vi "GV_SetGraph.vi"(8 "error in (no error)":errorcluster, 11 "Gviewer in":refnum<class "Gviewer.lvclass">) -> (0 "error out":errorcluster, 3 "Gviewer out":refnum<class "Gviewer.lvclass">)   [LabVIEW 2020, in "Sgraph_lib_V1.lvlib" / "Gviewer.lvclass"]
doc: "Set the Size and Position of the Graph"
uses:
  Gviewer.lvclass
  <vilib>/Utility/miscctls.llb/LVPositionTypeDef.ctl
  <vilib>/Utility/miscctls.llb/LVBoundsTypeDef.ctl
  Gviewer.lvclass/Gviewer.ctl
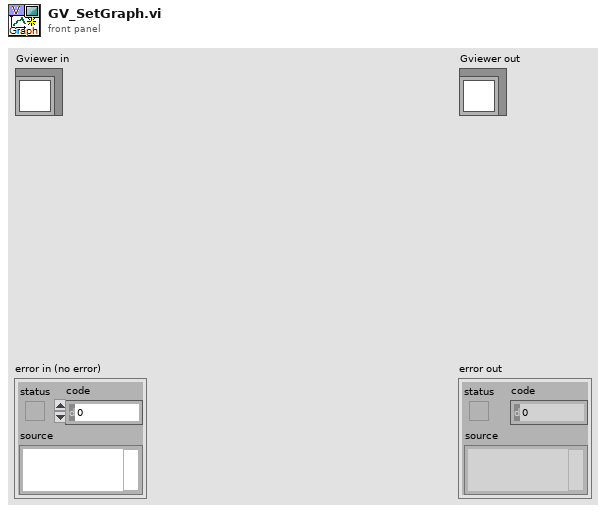
[diagram p1: front panel]
types:
  T1 = typedef "LVBoundsTypeDef.ctl" = cluster{"Width":u32, "Height":u32}
  T2 = typedef "LVPositionTypeDef.ctl" = cluster{"Left":i32, "Top":i32}
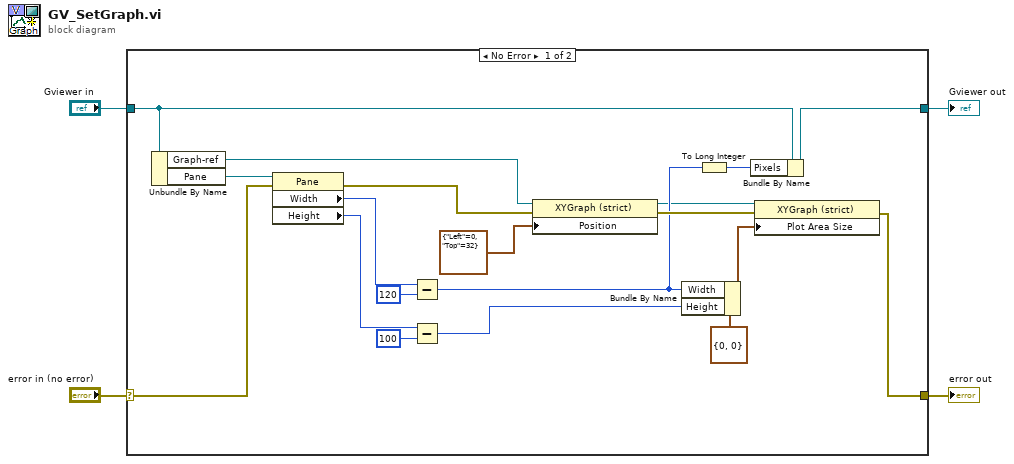
[diagram p0: block diagram]
diagram:
  n1 = case shown="No Error" "error in (no error)" {
    selector: "error in (no error)" -> [w19 w25]
    tunnel: [w17 w25] -> w3
    tunnel: [w10 w24] -> w1
    tunnel: "Gviewer in" -> [w7 w24]
    frame No Error {
      n2 = Unbundle By Name(w7) -> ("Graph-ref"=w5:refnum<vi>, "Pane"=w18:refnum<vi>)
      n3 = property class="Pane"(reference=w18, error in=w19) -> (error out=w6:errorcluster, "Width"=w21:u32, "Height"=w16:u32)  [unwired: 1 out]
      n4 = Subtract(x=w21, y=u32 120) -> (x-y=w11:u32)
      n5 = Subtract(x=w16, y=u32 100) -> (x-y=w14:u32)
      n6 = property class="XYGraph (strict)"(reference=w5, error in=w6, "Position"=T2 {"Left"=0, "Top"=32}) -> (reference out=w8:refnum<vi>, error out=w12:errorcluster)
      n7 = Bundle By Name(cluster=T1 {"Width"=0, "Height"=0} ("Draw Area Size"), "Width"=w11, "Height"=w14) -> (w13:T1)
      n8 = To Long Integer(number=w11) -> (32bit integer=w9:i32)
      n9 = Bundle By Name(cluster=w7, "Pixels"=w9) -> (w10:refnum<class "Gviewer.lvclass">)
      n10 = property class="XYGraph (strict)"(reference=w8, error in=w12, "Plot Area Size"=w13) -> (error out=w17:errorcluster)  [unwired: 1 out]
    }
    frame Error {
    }
  }
  "error out" <- w3
  "Gviewer out" <- w1
